vi "set Marker Frequency Count.vi"(6 "On?":bool, 8 "error in (no error)":errorcluster, 10 "Index":i32, 11 "Keysight 9020A in":refnum<class "Keysight 9020A.lvclass">) -> (0 "error out":errorcluster, 3 "Keysight 9020A out":refnum<class "Keysight 9020A.lvclass">)   [LabVIEW 2023, in "Spectrum Analyzer.lvlib" / "Keysight 9020A.lvclass"]
uses:
  Keysight 9020A.lvclass
  Keysight 9020A.lvclass/Keysight 9020A.ctl
  <vilib>/ErrorRing/Error Ring.xnode
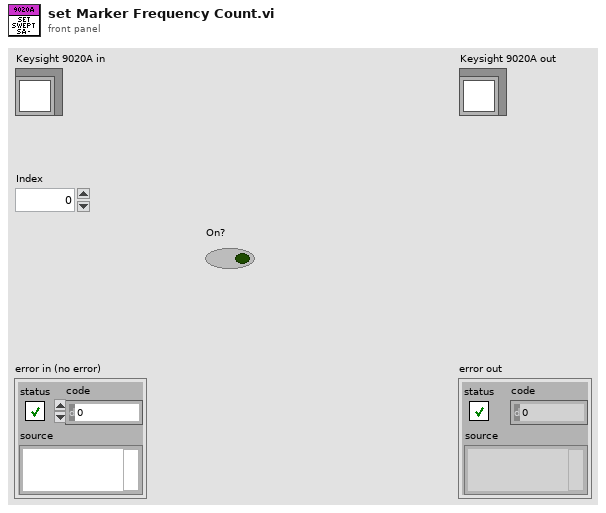
[diagram p1: front panel]
types:
  T1 = typedef "Spectrum Analyzer.lvlib/TYPE Measurement Preset.ctl" = enum16{"Sweep SA Mode", "Channel Power", "Occupied BW", "ACP", "Spurious Emission", "Spurious Emission Mask", "Burst Power (Transmit Power)"}
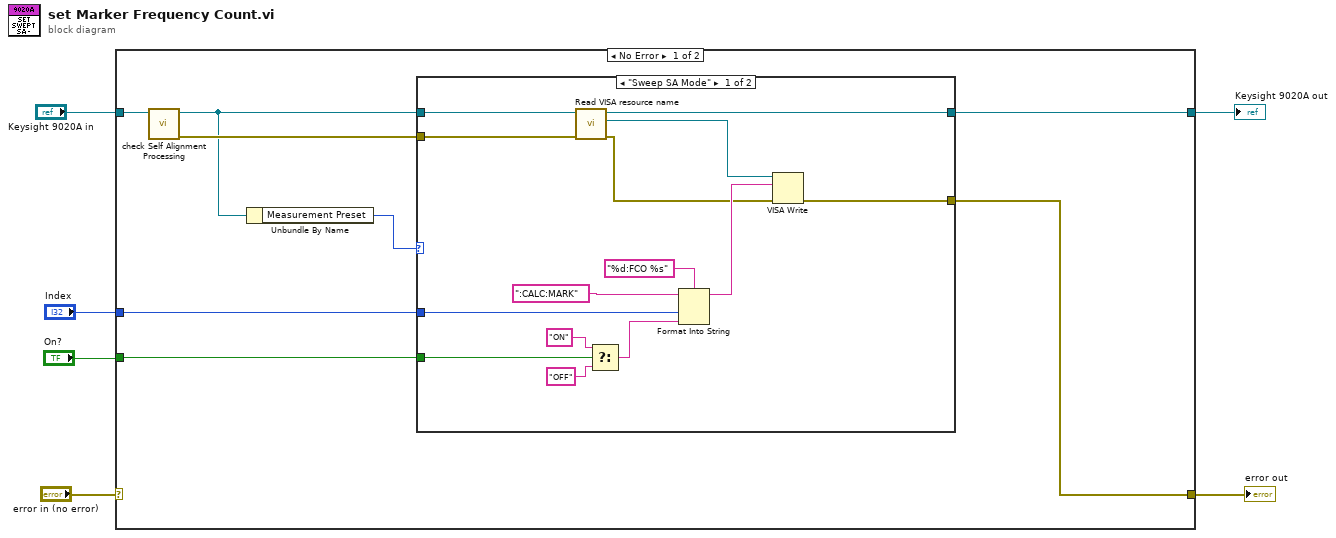
[diagram p0: block diagram]
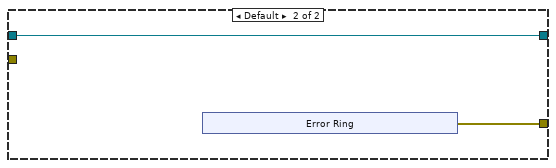
[diagram p2: hidden frame]
diagram:
  n1 = case shown="No Error" "error in (no error)" {
    selector: "error in (no error)" -> [_ w32]
    tunnel: "Keysight 9020A in" -> [w10 w33]
    tunnel: [w11 w33] -> w5
    tunnel: [w12 w32] -> w3
    tunnel: "Index" -> [w13 _]
    tunnel: "On?" -> [w14 _]
    frame No Error {
      n2 = call "check Self Alignment Processing.vi"("Keysight 9020A in"=w10) -> ("error out"=w9:errorcluster, "Keysight 9020A out"=w8:refnum<class "Keysight 9020A.lvclass">)  [unwired: 8 in, 1 out]
      n3 = Unbundle By Name(w8) -> ("Measurement Preset"=w7:T1)
      n4 = case shown="\"Sweep SA Mode\"" w7 {
        tunnel: w14 -> [w26 _]
        tunnel: w13 -> [w22 _]
        tunnel: [w21 w29] -> w12
        tunnel: [w19 w30] -> w11
        tunnel: w9 -> [w18 _]
        tunnel: w8 -> [w16 w30]
        frame "Sweep SA Mode" {
          n5 = call "Read VISA resource name.vi"("error in (no error)"=w18, "Keysight 9020A in"=w16) -> ("error out"=w17:errorcluster, "VISA resource name"=w20:refnum<visa-resource-name>, "Keysight 9020A out"=w19:refnum<class "Keysight 9020A.lvclass">)  [unwired: 7 in]
          n6 = Select(t="ON", s=w26, f="OFF") -> (s? t:f=w23:string)
          n7 = Format Into String(format string="%d:FCO %s", initial string=":CALC:MARK", w22, w23) -> (resulting string=w28:string)  [unwired: 1 in, 1 out]
          n8 = VISA Write(VISA resource name=w20, write buffer=w28, error in (no error)=w17) -> (error out=w21:errorcluster)  [unwired: 2 out]
        }
        frame Default {
          n9 = xnode "Error Ring"() -> ("error out"=w29:errorcluster)
        }
      }
    }
    frame Error {
    }
  }
  "error out" <- w3
  "Keysight 9020A out" <- w5
